vi "RT_Fault_Checker.vi"(8 "error in (no error)":errorcluster={"status"=FALSE, "code"=0, "source"="\"\""}, 10 "watchdog status":string, 11 "Sensor/controller status":string) -> (0 "error out":errorcluster={"status"=FALSE, "code"=0, "source"="\"\""}, 2 "status ok":bool, 3 "FaultRecord and protective request":string)   [LabVIEW 2026]
doc: "INTENT: Detect RT equipment and control faults. LOGIC: Evaluate overpressure, actuator error, invalid sensor and service loss independently of sequence wait state."
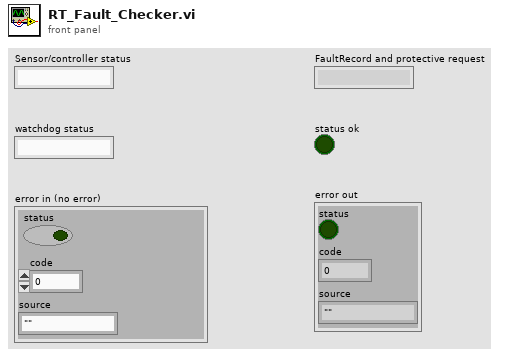
[diagram p1: front panel]
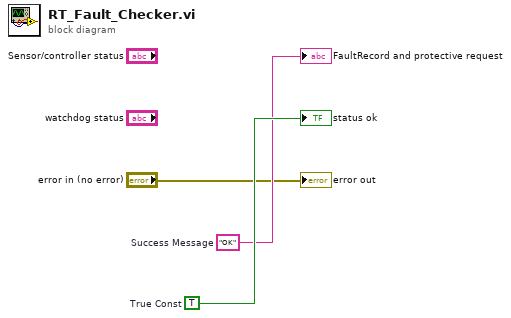
[diagram p0: block diagram]
diagram:
  w3 = TRUE  # True Const
  w2 = "OK"  # Success Message
  "FaultRecord and protective request" <- w2
  "status ok" <- w3
  "error out" <- "error in (no error)"
